vi "Check String Validity.vi"(4 "Regular Expression":string, 6 "String Name for Error":string, 9 "Max Characters":i32=-1, 10 "Valid String Specification":T1, 11 "String":string) -> (2 "string error":errorcluster, 3 "Valid":bool)   [LabVIEW 2015, in "NI_AWS_Core.lvlib" / "HTTP Request.lvclass"]
uses:
  HTTP Request.lvclass
  Valid String Specification.ctl
  <vilib>/regexp/Match Regular Expression.xnode
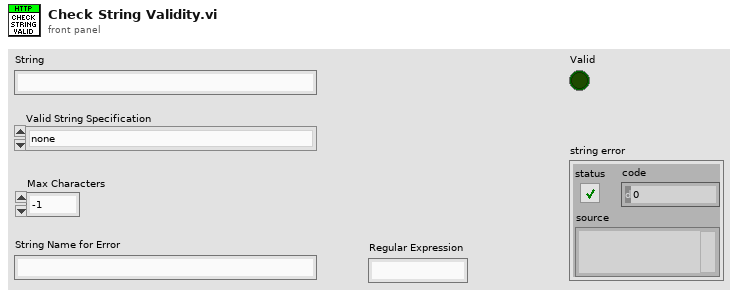
[diagram p1: front panel]
types:
  T1 = typedef "NI_AWS_Core.lvlib/HTTP Request.lvclass/Valid String Specification.ctl" = enum16{"none", "only [alphanumeric][-][_]", "only [alphanumeric][-][_][space]", "phone number +1xxxyyyzzzz", "Regular Expression"}
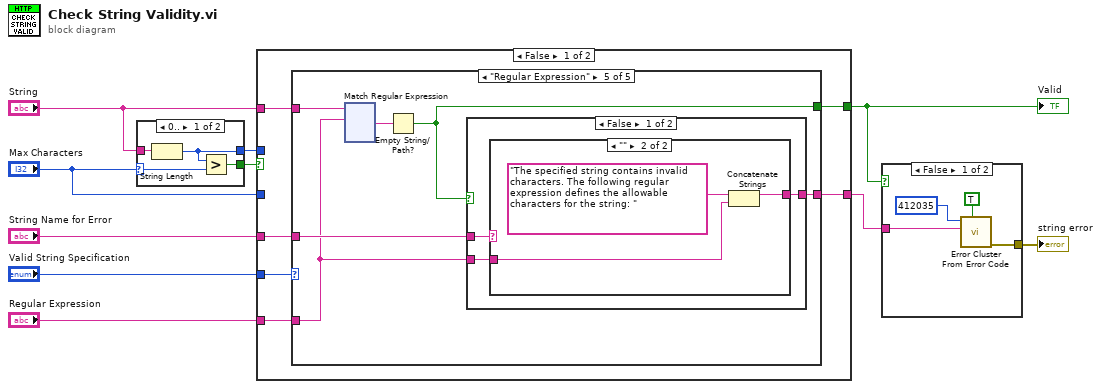
[diagram p0: block diagram]
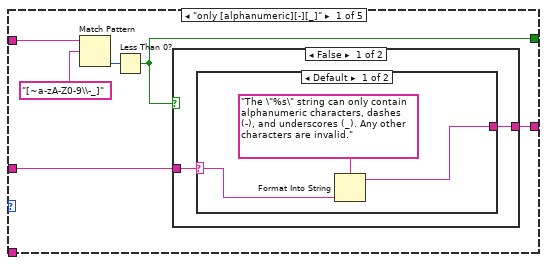
[diagram p4: hidden frame]
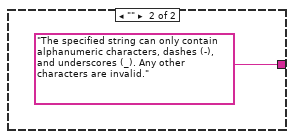
[diagram p5: hidden frame]
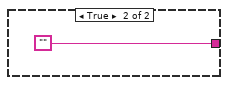
[diagram p6: hidden frame]
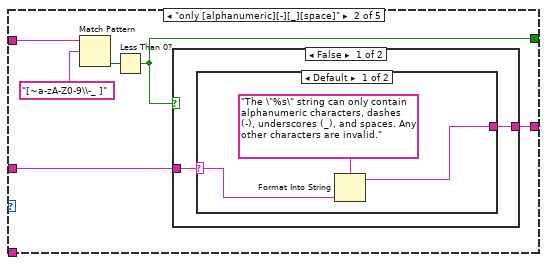
[diagram p7: hidden frame]
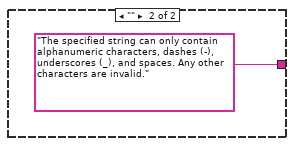
[diagram p8: hidden frame]
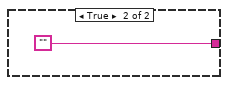
[diagram p9: hidden frame]
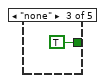
[diagram p10: hidden frame]
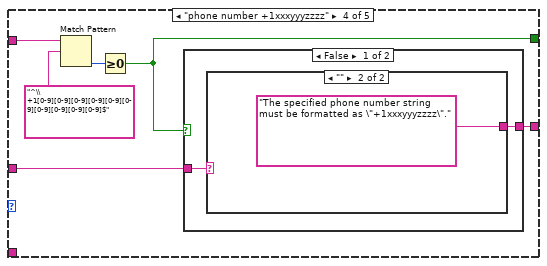
[diagram p11: hidden frame]
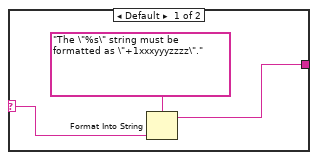
[diagram p12: hidden frame]
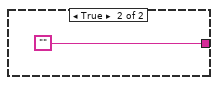
[diagram p13: hidden frame]
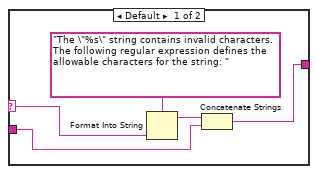
[diagram p14: hidden frame]
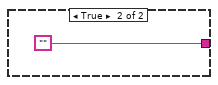
[diagram p15: hidden frame]
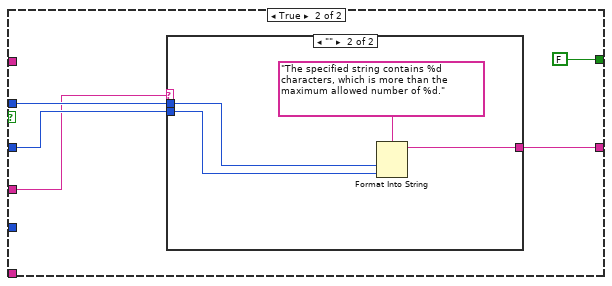
[diagram p16: hidden frame]
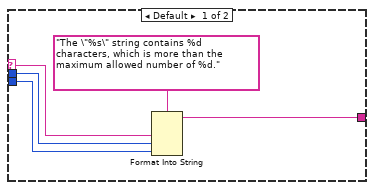
[diagram p17: hidden frame]
diagram:
  n1 = case shown="0.." "Max Characters" {
    selector: "Max Characters" -> [w12 _]
    tunnel: [w14 _] -> w10
    tunnel: "String" -> [w13 _]
    tunnel: [w11 _] -> w6
    frame 0.. {
      n2 = String Length(string=w13) -> (length=w11:i32)
      n3 = Greater?(x=w11, y=w12) -> (0:w14:bool)
    }
    frame ..-1 {
    }
  }
  n4 = case shown="False" w10 {
    tunnel: "String Name for Error" -> [w17 w194]
    tunnel: "String" -> [w19 _]
    tunnel: [w18 FALSE] -> w3
    tunnel: "Max Characters" -> [_ w195]
    tunnel: w6 -> [_ w196]
    tunnel: "Valid String Specification" -> [w20 _]
    tunnel: [w16 w193] -> w2
    tunnel: "Regular Expression" -> [w15 _]
    frame False {
      n5 = case shown="\"Regular Expression\"" w20 {
        tunnel: w19 -> [w26 w39 _ w51 w64]
        tunnel: [w22 w35 TRUE w48 w62] -> w18
        tunnel: w17 -> [w23 w36 _ w52 w65]
        tunnel: [w21 w34 _ w53 w66] -> w16
        tunnel: w15 -> [_ _ _ _ w61]
        frame "only [alphanumeric][-][_]" {
          n6 = Match Pattern(string=w26, regular expression="[~a-zA-Z0-9\\-_]") -> (offset past match=w24:i32)  [unwired: 1 in, 3 out]
          n7 = Less Than 0?(x=w24) -> (x < 0?=w22:bool)
          n8 = case shown="False" w22 {
            tunnel: w23 -> [w28 _]
            tunnel: [w27 ""] -> w21
            frame False {
              n9 = case shown="Default" w28 {
                selector: w28 -> [w30 _]
                tunnel: [w29 "The specified string can only contain alphanumeric characters, dashes (-), and underscores (_). Any other characters are invalid." ("error message (\"\")")] -> w27
                frame Default {
                  n10 = Format Into String(format string="The \"%s\" string can only contain alphanumeric characters, dashes (-), and underscores (_). Any other characters are invalid.", w30) -> (resulting string=w29:string)  [unwired: 2 in, 1 out]
                }
                frame "" {
                }
              }
            }
            frame True {
            }
          }
        }
        frame "only [alphanumeric][-][_][space]" {
          n11 = Match Pattern(string=w39, regular expression="[~a-zA-Z0-9\\-_ ]") -> (offset past match=w37:i32)  [unwired: 1 in, 3 out]
          n12 = Less Than 0?(x=w37) -> (x < 0?=w35:bool)
          n13 = case shown="False" w35 {
            tunnel: w36 -> [w41 _]
            tunnel: [w40 ""] -> w34
            frame False {
              n14 = case shown="Default" w41 {
                selector: w41 -> [w43 _]
                tunnel: [w42 "The specified string can only contain alphanumeric characters, dashes (-), underscores (_), and spaces. Any other characters are invalid." ("error message (\"\")")] -> w40
                frame Default {
                  n15 = Format Into String(format string="The \"%s\" string can only contain alphanumeric characters, dashes (-), underscores (_), and spaces. Any other characters are invalid.", w43) -> (resulting string=w42:string)  [unwired: 2 in, 1 out]
                }
                frame "" {
                }
              }
            }
            frame True {
            }
          }
        }
        frame "none" {
        }
        frame "phone number +1xxxyyyzzzz" {
          n16 = Match Pattern(string=w51, regular expression="^\\+1[0-9][0-9][0-9][0-9][0-9][0-9][0-9][0-9][0-9][0-9]$") -> (offset past match=w49:i32)  [unwired: 1 in, 3 out]
          n17 = Greater Or Equal To 0?(x=w49) -> (x >= 0?=w48:bool)
          n18 = case shown="False" w48 {
            tunnel: [w55 ""] -> w53
            tunnel: w52 -> [w54 _]
            frame False {
              n19 = case shown="\"\"" w54 {
                selector: w54 -> [w57 _]
                tunnel: [w56 "The specified phone number string must be formatted as \"+1xxxyyyzzzz\"." ("error message (\"\")")] -> w55
                frame Default {
                  n20 = Format Into String(format string="The \"%s\" string must be formatted as \"+1xxxyyyzzzz\".", w57) -> (resulting string=w56:string)  [unwired: 2 in, 1 out]
                }
                frame "" {
                }
              }
            }
            frame True {
            }
          }
        }
        frame "Regular Expression" {
          n21 = xnode "Match Regular Expression"("input string"=w64, "regular expression"=w61) -> ("after match"=w63:string)  [unwired: 4 in, 4 out]
          n22 = Empty String/Path?(string/path=w63) -> (empty?=w62:bool)
          n23 = case shown="False" w62 {
            tunnel: [w183 ""] -> w66
            tunnel: w65 -> [w182 _]
            tunnel: w61 -> [w181 _]
            frame False {
              n24 = case shown="\"\"" w182 {
                selector: w182 -> [w187 _]
                tunnel: [w185 w190] -> w183
                tunnel: w181 -> [w184 w189]
                frame Default {
                  n25 = Format Into String(format string="The \"%s\" string contains invalid characters. The following regular expression defines the allowable characters for the string: ", w187) -> (resulting string=w186:string)  [unwired: 2 in, 1 out]
                  n26 = Concatenate Strings(w186, w184) -> (w185:string)
                }
                frame "" {
                  n27 = Concatenate Strings("The specified string contains invalid characters. The following regular expression defines the allowable characters for the string: " ("error message (\"\")"), w189) -> (w190:string)
                }
              }
            }
            frame True {
            }
          }
        }
      }
    }
    frame True {
      n28 = case shown="\"\"" w194 {
        selector: w194 -> [w201 _]
        tunnel: w196 -> [w200 w203]
        tunnel: w195 -> [w199 w204]
        tunnel: [w198 w205] -> w193
        frame Default {
          n29 = Format Into String(format string="The \"%s\" string contains %d characters, which is more than the maximum allowed number of %d.", w201, w200, w199) -> (resulting string=w198:string)  [unwired: 2 in, 1 out]
        }
        frame "" {
          n30 = Format Into String(format string="The specified string contains %d characters, which is more than the maximum allowed number of %d.", w203, w204) -> (resulting string=w205:string)  [unwired: 2 in, 1 out]
        }
      }
    }
  }
  "Valid" <- w3
  n31 = case shown="False" w3 {
    tunnel: [w210 _] -> w4
    tunnel: w2 -> [w207 _]
    frame False {
      n32 = call <vilib>:"Error Cluster From Error Code.vi"("show call chain? (False)"=TRUE, "error message (\"\")"=w207, "error code (0)"=412035) -> ("error out"=w210:errorcluster)  [unwired: 6 in]
    }
    frame True {
    }
  }
  "string error" <- w4
